vi "VIH UI - Convert Pane Coords to Picture Control Coords.vi"(9 "Pane Coords":cluster{"Horizontal":i32, "Vertical":i32}, 11 "Pict Refnum":refnum<vi>) -> (1 "Picture Coords":cluster{"Horizontal":i32, "Vertical":i32}, 3 "dup Pict Refnum":refnum<vi>)   [LabVIEW 2014]
doc: "::: VI Helpeks :::\nCopyright (c) 2000-2026 Konstantin Shifershteyn. All rights reserved."
panel:
  # "VI Helpeks\nCopyright (c) 2012-2026 Konstantin Shifershteyn"
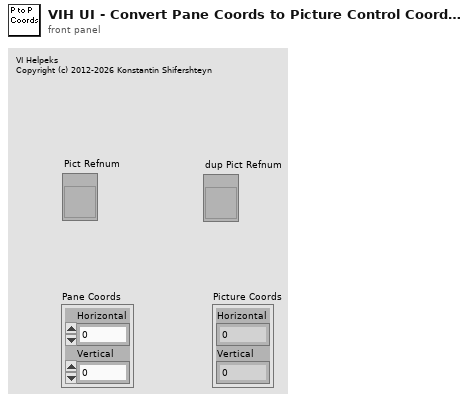
[diagram p1: front panel]
types:
  T1 = typedef "LVPositionTypeDef.ctl" = cluster{"Left":i32, "Top":i32}
  T2 = typedef "LVBoundsTypeDef.ctl" = cluster{"Width":u32, "Height":u32}
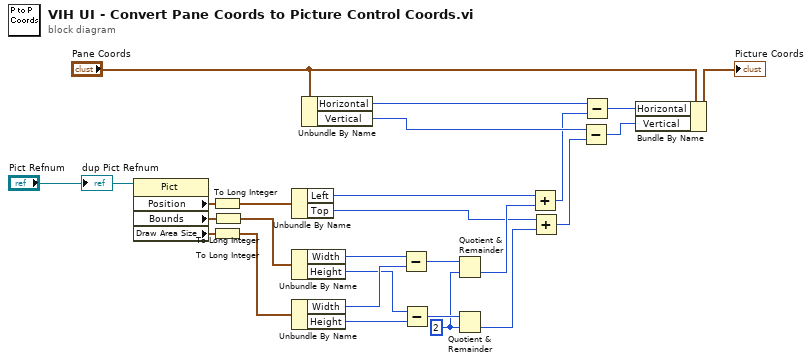
[diagram p0: block diagram]
diagram:
  w13 = 2 ("y")
  n1 = property class="Pict"(reference="Pict Refnum") -> ("Position"=w15:T1, "Bounds"=w24:T2, "Draw Area Size"=w25:T2)  [unwired: 1 in, 2 out]
  n2 = To Long Integer(number=w15) -> (32bit integer=w14:T1)
  n3 = To Long Integer(number=w25) -> (32bit integer=w17:cluster{"Width":i32, "Height":i32})
  n4 = To Long Integer(number=w24) -> (32bit integer=w16:cluster{"Width":i32, "Height":i32})
  n5 = Unbundle By Name(w14) -> ("Left"=w6:i32, "Top"=w5:i32)
  n6 = Unbundle By Name(w16) -> ("Width"=w23:i32, "Height"=w20:i32)
  n7 = Unbundle By Name(w17) -> ("Width"=w22:i32, "Height"=w21:i32)
  n8 = Unbundle By Name("Pane Coords") -> ("Horizontal"=w10:i32, "Vertical"=w9:i32)
  n9 = Subtract(x=w23, y=w22) -> (x-y=w19:i32)
  n10 = Subtract(x=w20, y=w21) -> (x-y=w18:i32)
  n11 = Quotient & Remainder(x=w19, y=w13) -> (floor(x/y)=w8:i32)  [unwired: 1 out]
  n12 = Quotient & Remainder(x=w18, y=w13) -> (floor(x/y)=w7:i32)  [unwired: 1 out]
  n13 = Add(x=w6, y=w8) -> (x+y=w4:i32)
  n14 = Add(x=w5, y=w7) -> (x+y=w3:i32)
  n15 = Subtract(x=w9, y=w3) -> (x-y=w1:i32)
  n16 = Subtract(x=w10, y=w4) -> (x-y=w2:i32)
  n17 = Bundle By Name(cluster="Pane Coords", "Horizontal"=w2, "Vertical"=w1) -> (→"Picture Coords":cluster{"Horizontal":i32, "Vertical":i32})
  "dup Pict Refnum" <- "Pict Refnum"
